vi "Native_CreateConstantFromTerminal_v2.vi"() -> ()   [LabVIEW 2024]
panel:
  out "error out":errorcluster caption="错误输出"
  out "created_terminal_id":u32
  in  "created_terminal_id type":u32
  out "constant_id":u32
  in  "constant_id type":u32
  in  "terminal_id":u32
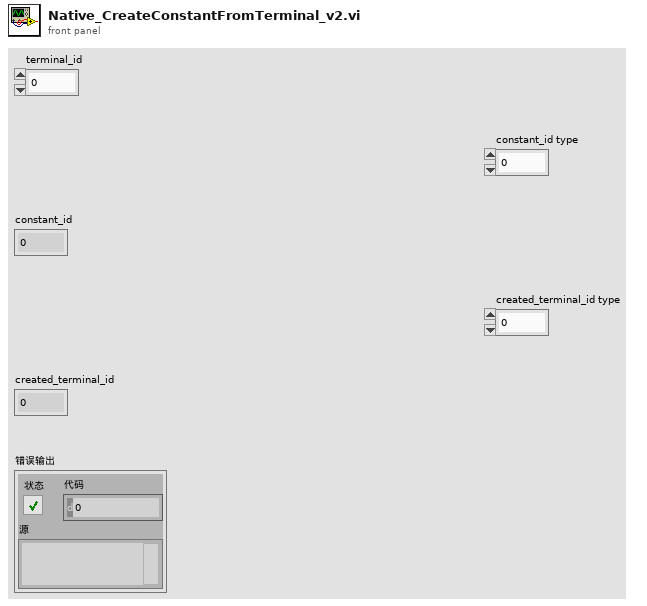
[diagram p1: front panel]
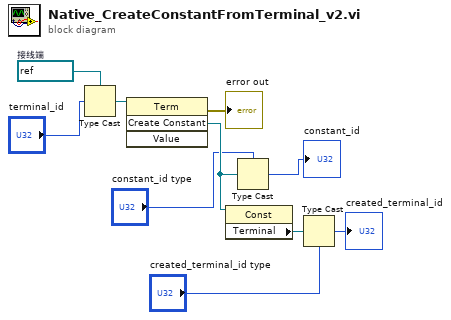
[diagram p0: block diagram]
diagram:
  w9 = refnum<vi> refnum  # 接线端
  n1 = Type Cast ("强制类型转换")(type=w9, x="terminal_id") -> (*(type *) &x=w8:refnum<vi>)
  n2 = invoke class="Term" method="Create Constant"(reference=w8) -> (error out=→"error out":errorcluster, "Create Constant"=w7:refnum<vi>)  [unwired: 3 in, 2 out]
  n3 = property on="属性节点" class="Const"(reference=w7) -> ("Terminal"=w4:refnum<vi>)  [unwired: 1 in, 2 out]
  n4 = Type Cast ("强制类型转换")(type="constant_id type", x=w7) -> (*(type *) &x=→"constant_id":u32)
  n5 = Type Cast ("强制类型转换")(type="created_terminal_id type", x=w4) -> (*(type *) &x=→"created_terminal_id":u32)
